vi "Virtual DAQ Signal erzeugen.vi"(0 "Physikalischer Kanal":string, 1 "Signalform":T1(ring), 2 "Frequenz Hz":dbl=50.0, 3 "Amplitude Vss":dbl=2.0, 4 "Offset V":dbl, 5 "Punkte pro Periode":i32=100, 6 "Spannungsbereich ±V":dbl=10.0) -> (20 "Signalvorschau":waveform(dbl)(graph), 21 "Status":dbl, 27 "error out":errorcluster)   [LabVIEW 2026]
doc: "Virtuelles SFP. Frequenz, Signalform, Spitze-Spitze und Offset in LabVIEW waehlen. Ein Lauf startet den gewaehlten Analogausgang. Ein neuer Lauf ersetzt das Signal auf dem gewaehlten Kanal."
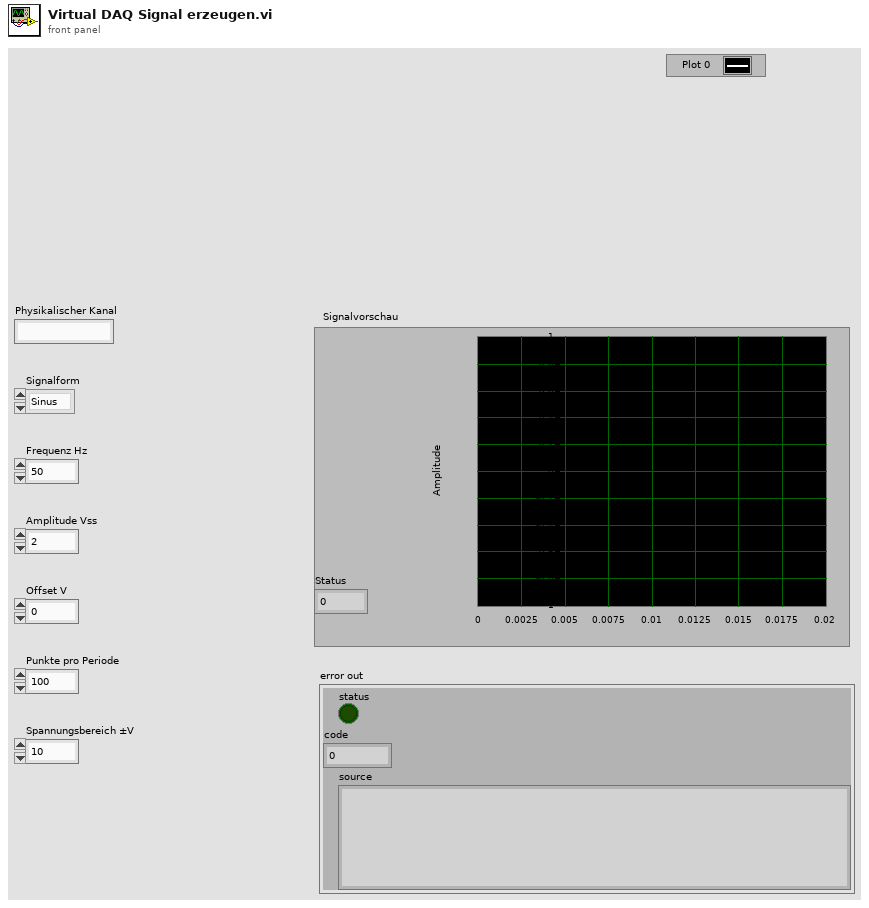
[diagram p1: front panel]
types:
  T1 = enum8{"Sinus", "Rechteck", "Dreieck", "Gleichspannung"}
  T2 = cluster{"Messart":enum8{"Wahl treffen", "AI Spannung", "AO Spannung", "DI Lesen", "DO Schreiben", "CTR Frequenz", "DMM Widerstand", "Ausgaenge freigeben"}, "Kanal":string, "PFI":string, "Rate":dbl, "Samples":i32, "Bereich":dbl, "Kontinuierlich":bool}
  T3 = enum8{"Wahl treffen", "AI Spannung", "AO Spannung", "DI Lesen", "DO Schreiben", "CTR Frequenz", "DMM Widerstand", "Ausgaenge freigeben"}
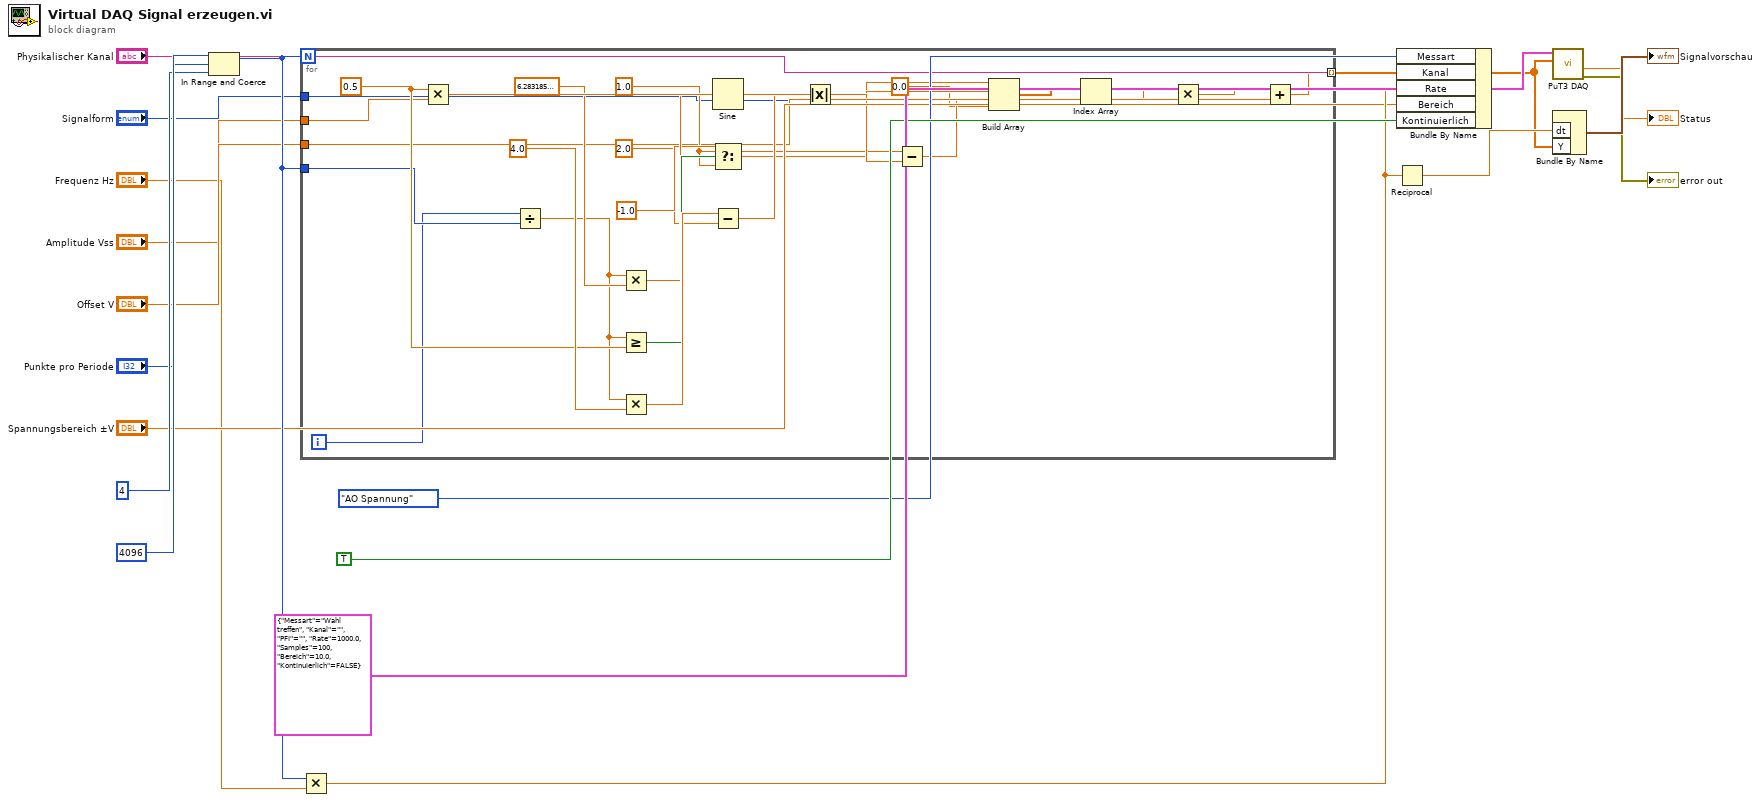
[diagram p0: block diagram]
diagram:
  n1 = In Range and Coerce(upper limit=4096, x="Punkte pro Periode", lower limit=4) -> (coerced(x)=w10:i32)  [unwired: 1 out]
  n2 = for {
    N: w10 -> [_]
    tunnel: "Signalform" -> [w24]
    tunnel: "Amplitude Vss" -> [w25]
    tunnel: "Offset V" -> [w26]
    tunnel: w10 -> [w22]
    tunnel: [w46] -> w11 mode=indexing
    i -> [w21]
    w31 = 0.5
    w28 = 1.0
    n3 = Multiply(x=w31, y=w25) -> (x*y=w44:dbl)
    n4 = Divide(x=w21, y=w22) -> (x/y=w23:dbl)
    n5 = Multiply(x=w23, y=6.283185307179586) -> (x*y=w33:dbl)
    n6 = Greater Or Equal?(x=w23, y=w31) -> (x >= y?=w35:bool)
    n7 = Multiply(x=w23, y=4.0) -> (x*y=w38:dbl)
    n8 = Sine(x=w33) -> (sin(x)=w34:dbl)
    n9 = Select(t=-1.0, s=w35, f=w28) -> (s? t:f=w36:dbl)
    n10 = Subtract(x=w38, y=2.0) -> (x-y=w39:dbl)
    n11 = Absolute Value(x=w39) -> (abs(x)=w40:dbl)
    n12 = Subtract(x=w28, y=w40) -> (x-y=w41:dbl)
    n13 = Build Array(w34, w36, w41, 0.0) -> (w42:dbl[])
    n14 = Index Array(array=w42, index=w24) -> (element=w43:dbl)
    n15 = Multiply(x=w43, y=w44) -> (x*y=w45:dbl)
    n16 = Add(x=w45, y=w26) -> (x+y=w46:dbl)
  }
  n17 = Multiply(x=w10, y="Frequenz Hz") -> (x*y=w12:dbl)
  n18 = Bundle By Name(cluster=T2 {"Messart"=enum."Wahl treffen", "Kanal"="", "PFI"="", "Rate"=1000.0, "Samples"=100, "Bereich"=10.0, "Kontinuierlich"=FALSE}, "Messart"=T3."AO Spannung", "Kanal"="Physikalischer Kanal", "Rate"=w12, "Bereich"="Spannungsbereich ±V", "Kontinuierlich"=TRUE) -> (w16:T2)
  n19 = Reciprocal(x=w12) -> (1/x=w19:dbl)
  n20 = call "PuT3 DAQ.vi"("Ausgabewerte"=w11, "Auftrag"=w16) -> ("error out"=→"error out":errorcluster, "Status"=→"Status":dbl)  [unwired: 6 in, 2 out]
  n21 = Bundle By Name("dt"=w19, "Y"=w11) -> (→"Signalvorschau":waveform(dbl))  [unwired: 1 in]
